vi "Save Project.vi"(6 "Project Active?":bool=TRUE, 7 "Project Store in":refnum<class "Project Store.lvclass">, 8 "error in":errorcluster, 9 "Task Names":string[](array[string]), 10 "Project Name":string, 11 "Project ID":string) -> (0 "error out":errorcluster, 3 "Project ID out":string, 5 "Project Store out":refnum<class "Project Store.lvclass">)   [LabVIEW 2026]
doc: "Adds a new project or updates an existing one, adds the tasks it does not have yet, and writes everything to the data source. An empty Project ID creates a new project (Add Project, which gives it a new GUID and the next Sort Order); otherwise the project's Name and Active are updated, and an unknown ID returns error 5102 (Save Project: project ID not found.). Every Task Name the project does not already have (exact name match, inactive tasks included) is added with Add Task - a new GUID, the next Sort Order, active. Existing tasks are left alone and nothing is removed; empty and repeated names are skipped.\n\nInputs: Project ID (empty for a new project); Project Name; Task Names; Project Active? (default TRUE); Project Store in; error in.\nOutputs: Project ID out; Project Store out; error out.\n\nGenerated by: Claude"
uses:
  Storage/Project Store/Project Store.lvclass
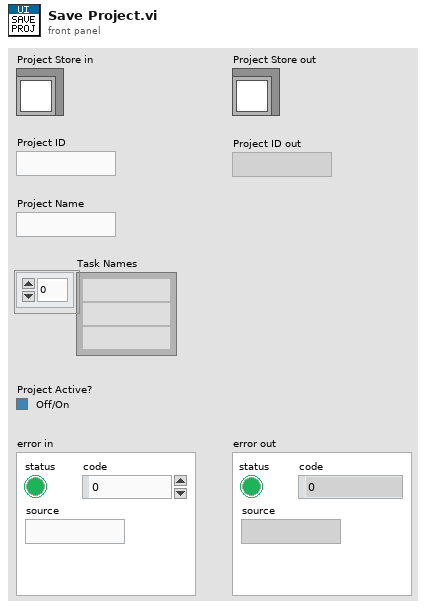
[diagram p1: front panel]
types:
  T1 = typedef "Project.ctl" = cluster{"ID":string, "Name":string, "Active":bool, "Sort Order":i32}
  T2 = typedef "Task List.ctl" = T3[]
  T3 = typedef "Task.ctl" = cluster{"ID":string, "Project ID":string, "Name":string, "Active":bool, "Sort Order":i32}
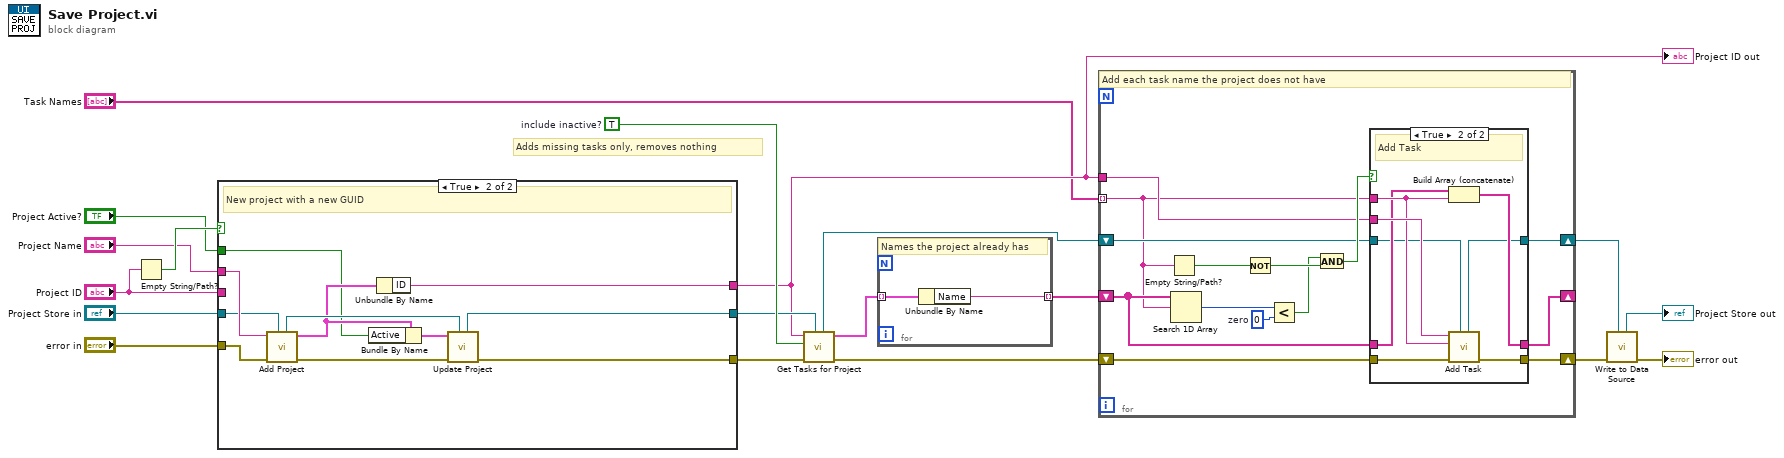
[diagram p0: block diagram]
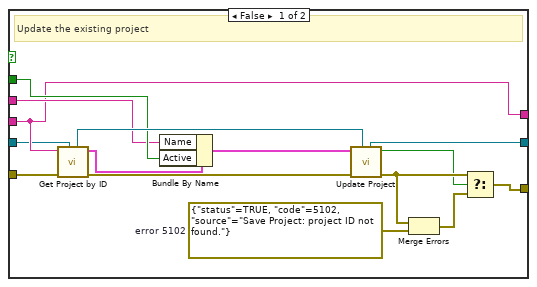
[diagram p3: hidden frame]
diagram:
  w13 = TRUE  # include inactive?
  # "Adds missing tasks only, removes nothing"
  n1 = Empty String/Path?(string/path="Project ID") -> (empty?=w10:bool)
  n2 = case shown="True" w10 {
    tunnel: "Project Store in" -> [w20 w35]
    tunnel: "error in" -> [w21 w36]
    tunnel: "Project ID" -> [w22 _]
    tunnel: "Project Name" -> [w23 w37]
    tunnel: "Project Active?" -> [w24 w38]
    tunnel: [w22 w45] -> w7
    tunnel: [w30 w43] -> w11
    tunnel: [w34 w44] -> w12
    frame False {
      w32 = errorcluster {"status"=TRUE, "code"=5102, "source"="Save Project: project ID not found."}  # error 5102
      # "Update the existing project"
      n3 = call-dynamic "Get Project by ID.vi"("Project Store in"=w20, "error in (no error)"=w21, "ID"=w22) -> ("error out"=w27:errorcluster, "Project"=w25:T1, "Project Store out"=w26:refnum<class "Project Store.lvclass">)  [unwired: 5 in, 1 out]
      n4 = Bundle By Name(cluster=w25, "Name"=w23, "Active"=w24) -> (w28:T1)
      n5 = call-dynamic "Update Project.vi"("Project Store in"=w26, "error in (no error)"=w27, "Project"=w28) -> ("error out"=w31:errorcluster, "found?"=w29:bool, "Project Store out"=w30:refnum<class "Project Store.lvclass">)  [unwired: 6 in]
      n6 = Merge Errors(w31, w32) -> (w33:errorcluster)
      n7 = Select(t=w31, s=w29, f=w33) -> (s? t:f=w34:errorcluster)
    }
    frame True {
      # "New project with a new GUID"
      n8 = call-dynamic "Add Project.vi"("Project Store in"=w35, "error in (no error)"=w36, "Name"=w37) -> ("error out"=w41:errorcluster, "Project"=w39:T1, "Project Store out"=w40:refnum<class "Project Store.lvclass">)  [unwired: 6 in]
      n9 = Bundle By Name(cluster=w39, "Active"=w38) -> (w42:T1)
      n10 = Unbundle By Name(w39) -> ("ID"=w45:string)
      n11 = call-dynamic "Update Project.vi"("Project Store in"=w40, "error in (no error)"=w41, "Project"=w42) -> ("error out"=w44:errorcluster, "Project Store out"=w43:refnum<class "Project Store.lvclass">)  [unwired: 6 in, 1 out]
    }
  }
  "Project ID out" <- w7
  n12 = call-dynamic "Get Tasks for Project.vi"("Project Store in"=w11, "error in (no error)"=w12, "include inactive?"=w13, "Project ID"=w7) -> ("error out"=w16:errorcluster, "Tasks"=w14:T2, "Project Store out"=w15:refnum<class "Project Store.lvclass">)  [unwired: 5 in]
  n13 = for {
    tunnel: w14 -> [w46] mode=indexing
    tunnel: [w47] -> w17 mode=indexing
    # "Names the project already has"
    n14 = Unbundle By Name(w46) -> ("Name"=w47:string)
  }
  n15 = for {
    tunnel: "Task Names" -> [w48] mode=indexing
    tunnel: w7 -> [w49]
    shift-right: [w51] -> w18
    shift-left: w15 -> [w50]
    shift-right: [w53] -> w19
    shift-left: w16 -> [w52]
    shift-right: [w55] -> _
    shift-left: w17 -> [w54]
    w56 = 0  # zero
    # "Add each task name the project does not have"
    n16 = Empty String/Path?(string/path=w48) -> (empty?=w59:bool)
    n17 = Search 1D Array(1D array=w54, element=w48) -> (index of element=w57:i32)  [unwired: 1 in]
    n18 = Not(x=w59) -> (.not. x?=w60:bool)
    n19 = Less?(x=w57, y=w56) -> (x < y?=w58:bool)
    n20 = And(x=w58, y=w60) -> (x .and. y?=w61:bool)
    n21 = case shown="True" w61 {
      tunnel: w48 -> [_ w68]
      tunnel: w49 -> [_ w69]
      tunnel: w50 -> [w62 w65]
      tunnel: w52 -> [w63 w66]
      tunnel: [w62 w70] -> w51
      tunnel: [w63 w71] -> w53
      tunnel: w54 -> [w64 w67]
      tunnel: [w64 w72] -> w55
      frame False {
        # "Already there or empty"
      }
      frame True {
        # "Add Task"
        n22 = Build Array (concatenate)(w67, w68) -> (w72:string[])
        n23 = call-dynamic "Add Task.vi"("Project Store in"=w65, "error in (no error)"=w66, "Name"=w68, "Project ID"=w69) -> ("error out"=w71:errorcluster, "Project Store out"=w70:refnum<class "Project Store.lvclass">)  [unwired: 5 in, 1 out]
      }
    }
  }
  n24 = call-dynamic "Write to Data Source.vi"("Project Store in"=w18, "error in (no error)"=w19) -> ("error out"=→"error out":errorcluster, "Project Store out"=→"Project Store out":refnum<class "Project Store.lvclass">)  [unwired: 8 in]
